vi "v6.vi"() -> ()   [LabVIEW 2025]
uses:
  <vilib>/Utility/miscctls.llb/LVDateTimeRec.ctl
  <vilib>/Platform/TimedLoop/XDataNode/timing_clust.ctl
  <vilib>/Platform/TimedLoop/XDataNode/nitl_modes.ctl
  <vilib>/Platform/TimedLoop/XDataNode/wakeup.ctl
  <vilib>/Analysis/3filter.llb/Filter Passband Type.ctl
  <vilib>/Instr/_visa.llb/VISA Configure Serial Port (Instr).vi
  <vilib>/Utility/inputDevices.llb/mouseAcquire.vi
  <vilib>/Analysis/3filter.llb/Butterworth Filter (DBL).vi
  <vilib>/Utility/file.llb/Write Delimited Spreadsheet (DBL).vi
  <vilib>/platform/TimedLoop/XDataNode/XDataNode.xnode
  <vilib>/Platform/TimedLoop/XDataNode/XDNodeRunTimeDep.lvlib
  <vilib>/Analysis/NI_AALPro.lvlib
  <vilib>/Analysis/NI_AALBase.lvlib
panel:
  out "erro_graus":dbl
  out "PV":dbl
  out "erro_abs_graus":dbl
  out "p_final":dbl
  out "array_frame_mov":i32[](array[numeric])
  out "array_mov":dbl[](array[numeric])
  out "TM_escre":string
  out "TM":i32
  out "ref":dbl
  out "velocidadepx":dbl[](array[numeric])
  out "referencia de endereco":path
  out "frames":i32[](array[numeric])
  out "TR":i32
  out "px_posicao":dbl[](array[numeric])
  out "t_max":dbl
  out "intervalo_preparacao":dbl
  out "intervalo_TR":dbl
  out "Vertical (cm/px)":dbl
  out "Horizontal (cm/px)":dbl
  out "INICIO_Cluter":T1
  out "INICIO":dbl format="%#.10g"
  out "ref_V_alvo":dbl
  out "ref_H_alvo":dbl
  out "ref_pont":dbl
  out "tentativa":i32
  out "cursor":picture
  in  "Tab Control":enum32{"Execucao", "Configuração"}(tab)
  out "tela":picture
  in  "Cor do ponteiro":u32(colorbox)=14421504
  in  "Cor_home":u32(colorbox)=197379
  in  "Horizontal (px)":dbl=1920.0
  in  "Horizontal (cm)":dbl=34.5
  in  "Raio_home":dbl=0.8
  in  "Horizontal_home":dbl=17.23
  in  "Vertical_home":dbl=20.0
  in  "Tamanho do ponteiro":dbl=0.3
  in  "Sincronizar com EEG":bool
  in  "Número de tentativas":i32=40
  in  "Digite aqui o endereço e nome do arquivo":string="C:\\bryan\\"
  in  "Vertical  (cm)":dbl=19.0
  in  "Vertical (px)":dbl=1080.0 format="%#_13g"
  in  "Horizontal_1":dbl=17.23
  in  "Vertical_1":dbl=23.0
  in  "Raio_1":dbl=0.5
  in  "Cor_1":u32(colorbox)=16775513
  in  "PORTA COM":refnum<visa-resource-name>
  in  "menor":dbl=2000.0 format="%#_13g"
  in  "preparacao 2":dbl=2000.0 format="%#_13g"
  in  "Tempo max  para fechar a tarefa":dbl=1500.0
  in  "FB":dbl=3000.0 format="%#_13g"
  in  "meta_tempo":dbl=250.0 format="%#_13g"
  out "home":picture
  # "100 h\n500 v"
  # "800 h\n100 v"
  # "Intervalo entre o prepara e vai"
  # "Tempo de preparação"
  # "Tempo de Feedback"
  # "Meta tempo"
  # "Home"
  # "Ponteiro"
  # "Para saber quantos cm preciso para um valor determinado de graus a percorre\n\n1. Divida o tamanho da tela vertical por 380 (ex.,19/380 = 0,05);\n2. Multiplique esse resultado pelo angulo de interesse (ex., 0,05*60 =3)"
  # "Posição do alvo"
  # "Horizontal"
  # "Raio"
  # "Vertical"
  # "Desenvolvido por Tércio Apolinário-Souza"
  # "Variability"
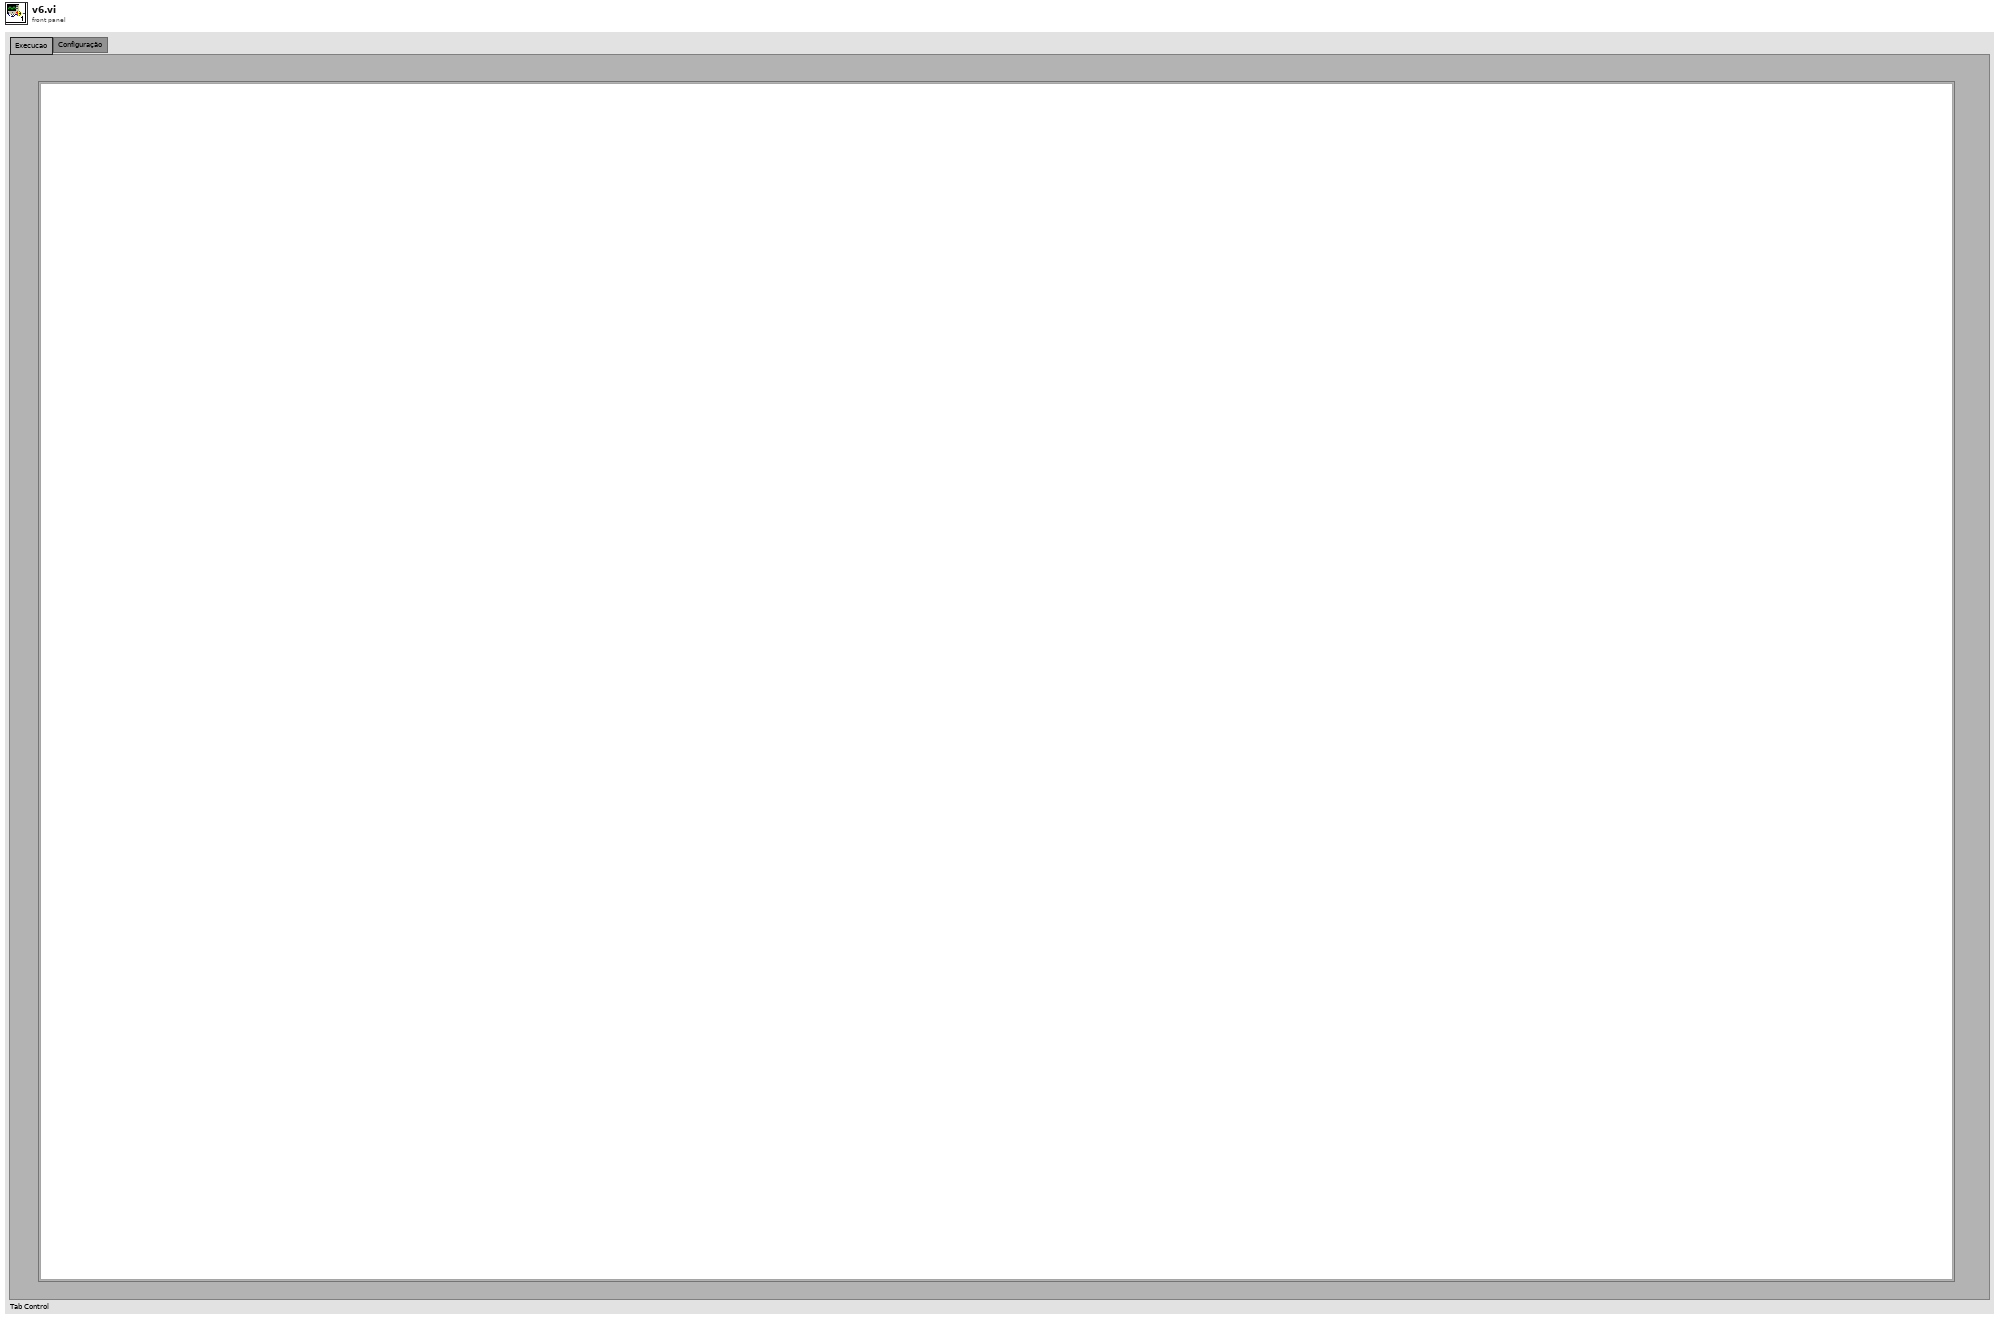
[diagram p1: front panel]
types:
  T1 = typedef "LVDateTimeRec.ctl" = cluster{"fractional second":dbl, "second":i32, "minute":i32, "hour":i32, "day of month":i32, "month":i32, "year":i32, "day of week":i32, "day of year":i32, "DST":i32}
  T2 = typedef "XDNodeRunTimeDep.lvlib/timing_clust.ctl" = cluster{"Expected End [f-1]":u64, "Actual End [f-1]":u64, "Finished Late? [f-1]":bool, "Expected End [i-1]":u64, "Actual End [i-1]":u64, "Finished Late? [i-1]":bool, "Expected Start [i]":u64, "Actual Start [i]":u64, "Expected Start [f]":u64, "Actual Start [f]":u64, "Source Name":string, "Structure Name":string, "Period":i64, "Deadline":i64, "Offset":i64, "Start":i64, "Priority":i32, "Timeout":i32, "Mode":T3, "Wakeup Reason":T4, "Error":errorcluster, "Source Type":string, "Secondary Source Type":string, "Global End Time":u64, "Global Start Time":u64, "Frame Duration":u64, "Iteration Duration":u64, "Assigned CPU":i32, "I/O Scan Engine Mode":u32}
  T3 = typedef "XDNodeRunTimeDep.lvlib/nitl_modes.ctl" = enum32{"No Change", "Process missed periods, maintain original phase", "Discard missed periods, maintain original phase", "Process missed periods, ignore original phase", "Discard missed periods, ignore original phase"}
  T4 = typedef "XDNodeRunTimeDep.lvlib/wakeup.ctl" = enum32{"Normal", "Aborted", "Asynchronous wakeup", "Timing source error", "Timed loop error", "Timeout"}
  T5 = typedef "NI_AALBase.lvlib/Filter Passband Type.ctl" = enum32{"Lowpass", "Highpass", "Bandpass", "Bandstop"}
  T6 = cluster{"button 1":bool, "button 2":bool, "button 3":bool, "button 4":bool}
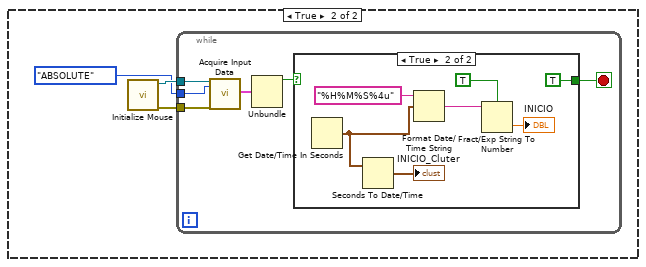
[diagram p2: hidden frame]
diagram:
  # "esquerda\ncima\ndireita\nbaixo"
  n1 = VISA Open(VISA resource name="PORTA COM") -> (VISA resource name=w21:refnum<visa-resource-name>, error out=w20:errorcluster)  [unwired: 4 in]
  n2 = VISA Close(VISA resource name=w21, error in (no error)=w20) -> (error out=w19:errorcluster)
  n3 = VISA Open(error in (no error)=w19, VISA resource name=w21) -> (VISA resource name=w18:refnum<visa-resource-name>, error out=w15:errorcluster)  [unwired: 3 in]
  n4 = for {
    N: "Número de tentativas" -> [_]
    tunnel: w18 -> [w38]
    tunnel: u32 9600 ("baud rate (9600)") -> [w37]
    tunnel: u16 8 ("data bits (8)") -> [w36]
    tunnel: w15 -> [w35]
    tunnel: [w30] -> w10 mode=indexing
    tunnel: [w29] -> w8 mode=indexing
    tunnel: [w28] -> w6 mode=indexing
    tunnel: [w27] -> w4 mode=indexing
    tunnel: [w26] -> w3 mode=indexing
    i -> [w40]
    n5 = call-poly "VISA Configure Serial Port"("VISA resource name"=w38, "baud rate (9600)"=w37, "data bits (8)"=w36, "error in (no error)"=w35) -> ("VISA resource name out"=w34:refnum<visa-resource-name>, "error out"=w33:errorcluster)  [unwired: 10 in]
    n6 = Increment(x=w40) -> (x+1=→"tentativa":i32)
    n7 = flat-sequence {
      tunnel: w40 -> [w44]
      tunnel: w34 -> [w42]
      tunnel: w33 -> [w43]
      tunnel: [w43] -> w32
      tunnel: [w42] -> w31
      tunnel: w32 -> [w74]
      tunnel: w31 -> [w75]
      tunnel: [w75] -> w25
      tunnel: [w74] -> w24
      tunnel: w25 -> [w94]
      tunnel: w24 -> [w93]
      tunnel: [w304] -> w30
      tunnel: [w301] -> w29
      tunnel: [w295] -> w28
      tunnel: [w290] -> w27
      tunnel: [w285] -> w26
      frame #0 {
        n8 = property on="TM_escre" class="Str"("Visible"=FALSE) -> ()  [unwired: 2 in, 2 out]
        n9 = Equal?(x=w44, y=0) -> (x = y?=w48:bool)
        n10 = And(x="Sincronizar com EEG", y=w48) -> (x .and. y?=w46:bool)
        n11 = case shown="False" w46 {
          frame False {
          }
          frame True {
            n12 = call <vilib>:"Initialize Mouse.vi"() -> ("error out"=w50:errorcluster, "device ID"=w51:refnum<k1>)  [unwired: 10 in]
            n13 = while {
              tunnel: w51 -> [w57]
              tunnel: w50 -> [w56]
              tunnel: enum16{"RELATIVE", "ABSOLUTE"}."ABSOLUTE" ("key mode") -> [w55]
              stop <- w53 stop-if-true
              n14 = call-poly <vilib>:"Acquire Input Data.vi"("device ID"=w57, "key mode"=w55, "error in (no error)"=w56) -> ("button info"=w54:T6)  [unwired: 13 in, 3 out]
              n15 = Unbundle(w54) -> ("button 1"=w52:bool)  [unwired: 3 out]
              n16 = case shown="True" w52 {
                tunnel: [_ TRUE] -> w53
                frame False {
                }
                frame True {
                  n17 = Get Date/Time In Seconds() -> (seconds since 1Jan1904=w59:timestamp)
                  n18 = Seconds To Date/Time(time stamp (now)=w59) -> (date time rec=→"INICIO_Cluter":T1)  [unwired: 1 in]
                  n19 = Format Date/Time String(time format string (%c)="%H%M%S%4u", seconds (now)=w59) -> (date/time string=w61:string)  [unwired: 1 in]
                  n20 = Fract/Exp String To Number(use system decimal point (T)=TRUE, string=w61) -> (number=→"INICIO":dbl)  [unwired: 2 in, 1 out]
                }
              }
            }
          }
        }
      }
      frame #1 {
        n21 = Quotient & Remainder(x="menor", y=5.0) -> (floor(x/y)=→"intervalo_TR":dbl)  [unwired: 1 out]
        n22 = Quotient & Remainder(x="preparacao 2", y=5.0) -> (floor(x/y)=→"intervalo_preparacao":dbl)  [unwired: 1 out]
        n23 = Divide(x="Vertical  (cm)", y="Vertical (px)") -> (x/y=→"Vertical (cm/px)":dbl)
        n24 = Divide(x="Horizontal (cm)", y="Horizontal (px)") -> (x/y=→"Horizontal (cm/px)":dbl)
        n25 = Quotient & Remainder(x="Tempo max  para fechar a tarefa", y=5.0) -> (floor(x/y)=→"t_max":dbl)  [unwired: 1 out]
      }
      frame #2 {
        n26 = node-c288(i64 5 ("Period")) -> (w92:T2)  [unwired: 3 in]
        n27 = timed-loop {
          tunnel: w94 -> [w152]
          tunnel: w93 -> [w151]
          timing: w92 -> [_]
          timing-out: [_] -> w91
          tunnel: [w144] -> w87
          tunnel: [w143] -> w86
          shift-right: [w124] -> w82
          shift-left: dbl[] [0.0] -> [w123]
          shift-right: [w122] -> w83
          shift-left: i32[] [0] -> [w121]
          i -> [w111]
          stop <- w145 stop-if-true
          # "Alvo"
          n28 = node-c288() -> ()  [unwired: 1 in, 1 out]
          n29 = VISA Read(VISA resource name=w152, byte count=u32 300, error in (no error)=w151) -> (VISA resource name out=w144:refnum<visa-resource-name>, read buffer=w153:string, error out=w143:errorcluster)  [unwired: 1 out]
          n30 = local read "Vertical_home"() -> (w142:dbl)
          n31 = local read "Vertical  (cm)"() -> (w169:dbl)
          n32 = local read "intervalo_TR"() -> (w128:dbl)
          n33 = local read "intervalo_preparacao"() -> (w119:dbl)
          n34 = local read "Horizontal (cm/px)"() -> (w161:dbl)
          n35 = local read "Horizontal_home"() -> (w141:dbl)
          n36 = local read "intervalo_TR"() -> (w120:dbl)
          n37 = local read "Raio_home"() -> (w140:dbl)
          n38 = local read "intervalo_preparacao"() -> (w106:dbl)
          n39 = local read "intervalo_preparacao"() -> (w126:dbl)
          n40 = local read "intervalo_preparacao"() -> (w131:dbl)
          n41 = local read "t_max"() -> (w129:dbl)
          n42 = Subtract(x=w169, y=w142) -> (x-y=w168:dbl)
          n43 = local read "intervalo_TR"() -> (w130:dbl)
          n44 = Spreadsheet String To Array(delimiter (Tab)=",", format string="%f", spreadsheet string=w153, array type (2D Dbl)=dbl[] []) -> (array=w154:dbl[])
          n45 = Add(x=w129, y=w128) -> (x+y=w127:dbl)
          n46 = Divide(x=w140, y=w161) -> (x/y=w166:dbl)
          n47 = Divide(x=w141, y=w161) -> (x/y=w171:dbl)
          n48 = Divide(x=w168, y=w161) -> (x/y=w146:dbl)
          n49 = Add(x=w120, y=w119) -> (x+y=w116:dbl)
          n50 = local read "Vertical  (cm)"() -> (w170:dbl)
          n51 = local read "Cor_home"() -> (w136:u32)
          n52 = local read "Vertical_1"() -> (w163:dbl)
          n53 = local read "Horizontal (cm/px)"() -> (w176:dbl)
          n54 = Add(x=w126, y=w127) -> (x+y=w125:dbl)
          n55 = Add(x=w131, y=w130) -> (x+y=w132:dbl)
          n56 = Index Array(array=w154) -> (element=w98:dbl)  [unwired: 1 in]
          n57 = Bundle(w171, w146) -> (w175:cluster{dbl, dbl})  [unwired: 1 in]
          n58 = Add(x=w116, y=2.0) -> (x+y=w115:dbl)
          n59 = Add(x=w106, y=2.0) -> (x+y=w110:dbl)
          n60 = local read "Horizontal_1"() -> (w165:dbl)
          n61 = Greater?(x=w111, y=w116) -> (0:w117:bool)
          n62 = Less?(x=w111, y=w115) -> (x < y?=w114:bool)
          n63 = Greater?(x=w111, y=w106) -> (0:w108:bool)
          n64 = Less?(x=w111, y=w110) -> (x < y?=w107:bool)
          n65 = Equal?(x=w125, y=w111) -> (x = y?=w145:bool)
          n66 = Greater?(x=w111, y=w131) -> (0:w134:bool)
          n67 = Less?(x=w111, y=w132) -> (x < y?=w133:bool)
          n68 = Subtract(x=w170, y=w163) -> (x-y=w167:dbl)
          n69 = Insert Into Array(array=w121, new element=w111) -> (w122:i32[])  [unwired: 1 in]
          n70 = Multiply(x=360.0, y=w98) -> (x*y=w149:dbl)
          n71 = And(x=w134, y=w133) -> ()  [unwired: 1 out]
          n72 = local read "Raio_1"() -> (w164:dbl)
          n73 = And(x=w117, y=w114) -> (x .and. y?=w113:bool)
          n74 = And(x=w108, y=w107) -> (x .and. y?=w109:bool)
          n75 = call <vilib>:"Draw Circle by Radius.vi"("color(black)"=w136, "fill?(F)"=TRUE, "pixel center"=w175, "radius"=w166) -> ("new picture"=w137:picture)  [unwired: 7 in]
          n76 = Divide(x=w165, y=w176) -> (x/y=w160:dbl)
          "ref_H_alvo" <- w160
          n77 = Divide(x=w167, y=w176) -> (x/y=w159:dbl)
          "ref_V_alvo" <- w159
          n78 = Divide(x=w149, y=1024.0) -> (x/y=w96:dbl)
          n79 = case shown="True" w113 {
            frame False {
            }
            frame True {
              # "Imperatus"
              n80 = call <vilib>:"Beep.vi"("use system alert? (T)"=FALSE, "duration (msec)"=u32 200, "frequency (Hz)"=u32 700) -> ()  [unwired: 9 in]
            }
          }
          n81 = case shown="True" w109 {
            frame False {
            }
            frame True {
              # "Warning"
              n82 = call <vilib>:"Beep.vi"("use system alert? (T)"=FALSE, "duration (msec)"=u32 200, "frequency (Hz)"=u32 500) -> ()  [unwired: 9 in]
            }
          }
          n83 = local write "home"(w137) -> ()
          n84 = Divide(x=w164, y=w176) -> (x/y=w178:dbl)
          n85 = local read "Horizontal (px)"() -> (w104:dbl)
          n86 = local read "Vertical (px)"() -> (w105:dbl)
          n87 = local read "Tamanho do ponteiro"() -> (w139:dbl)
          n88 = local read "Horizontal (cm/px)"() -> (w173:dbl)
          n89 = Bundle(w160, w159) -> (w99:cluster{dbl, dbl})  [unwired: 1 in]
          n90 = Divide(x=w96, y=380.0) -> (x/y=w97:dbl)
          n91 = local read "Cor_1"() -> (w162:u32)
          n92 = local read "Cor do ponteiro"() -> (w135:u32)
          n93 = Multiply(x=w97, y=w105) -> (x*y=w95:dbl)
          n94 = Quotient & Remainder(x=w104, y=2.0) -> (floor(x/y)=w102:dbl)  [unwired: 1 out]
          n95 = Divide(x=w139, y=w173) -> (x/y=w172:dbl)
          "ref_pont" <- w172
          n96 = Insert Into Array(array=w123, new element=w95) -> (w124:dbl[])  [unwired: 1 in]
          n97 = call <vilib>:"Draw Circle by Radius.vi"("color(black)"=w162, "fill?(F)"=TRUE, "pixel center"=w99, "radius"=w178, "picture"=w137) -> ("new picture"=w138:picture)  [unwired: 6 in]
          n98 = Bundle(w102, w95) -> (w180:cluster{dbl, dbl})  [unwired: 1 in]
          n99 = local write "cursor"(w138) -> ()
          n100 = call <vilib>:"Draw Circle by Radius.vi"("color(black)"=w135, "fill?(F)"=TRUE, "pixel center"=w180, "radius"=w172, "picture"=w138) -> ("new picture"=w100:picture)  [unwired: 6 in]
          n101 = call <vilib>:"Draw Circle by Radius.vi"("picture"=w100) -> ("new picture"=w101:picture)  [unwired: 10 in]
          n102 = local write "tela"(w101) -> ()
          n103 = node-c288() -> ()  [unwired: 1 in, 1 out]
        }
        "px_posicao" <- w82
        "frames" <- w83
        n104 = node-c288(w91) -> ()  [unwired: 1 out]
        n105 = VISA Clear(VISA resource name=w87, error in (no error)=w86) -> (VISA resource name out=w89:refnum<visa-resource-name>, error out=w88:errorcluster)
        n106 = VISA Close(VISA resource name=w89, error in (no error)=w88) -> ()  [unwired: 1 out]
      }
      frame #3 {
        # "Filtro"
        # "Filtro"
        n107 = call <vilib>:"Draw Circle by Radius.vi"() -> ("new picture"=w213:picture)  [unwired: 11 in]
        n108 = local write "tela"(w213) -> ()
        n109 = local read "px_posicao"() -> (w200:dbl[])
        n110 = Wait (ms)(milliseconds to wait=u32 10) -> ()  [unwired: 1 out]
        n111 = call-poly <vilib>:"Butterworth Filter.vi"("order"=2, "filter type"=Filter_Passband_Type."Lowpass", "low cutoff freq: fl"=12.0, "sampling freq: fs"=200.0, "X"=w200) -> ("Filtered X"=w208:dbl[])  [unwired: 3 in, 1 out]
        n112 = call <vilib>:"Derivative x(t).vi"("dt"=0.01, "Initial Condition"=dbl[] [0.0], "X"=w208) -> ("dX/dt"=w201:dbl[])  [unwired: 7 in, 1 out]
        n113 = call-poly <vilib>:"Butterworth Filter.vi"("order"=2, "filter type"=Filter_Passband_Type."Lowpass", "low cutoff freq: fl"=12.0, "sampling freq: fs"=100.0, "X"=w201) -> ("Filtered X"=w195:dbl[])  [unwired: 3 in, 1 out]
        n114 = Array Size(array=w195) -> (size(s)=w198:i32)
        n115 = Subtract(x=w198, y=1) -> (x-y=w196:i32)
        n116 = Array Subset(array=w195, index=0, length=w196) -> (→"velocidadepx":dbl[])
      }
      frame #4 {
        n117 = while {
          tunnel: [w220] -> w215
          tunnel: [w217] -> w216
          i -> [w220]
          stop <- w218 stop-if-true
          n118 = local read "intervalo_preparacao"() -> (w225:dbl)
          n119 = local read "velocidadepx"() -> (w227:dbl[])
          n120 = local read "intervalo_TR"() -> (w226:dbl)
          n121 = Add(x=w226, y=w225) -> (x+y=w217:dbl)
          n122 = Array Size(array=w227) -> (size(s)=w219:i32)
          n123 = Array Subset(array=w227, index=w217, length=w219) -> (w224:dbl[])
          n124 = Absolute Value(x=w224) -> (abs(x)=w223:dbl[])
          n125 = Greater?(x=w220, y=w219) -> (0:w221:bool)
          n126 = Index Array(array=w223, index=w220) -> (element=w231:dbl)
          n127 = Array Max & Min(array=w223) -> (max value=w230:dbl)  [unwired: 3 out]
          "PV" <- w230
          n128 = Multiply(x=w230, y=0.2) -> (x*y=w228:dbl)
          "ref" <- w228
          n129 = Greater?(x=w231, y=w228) -> (0:w222:bool)
          n130 = Or(x=w222, y=w221) -> (x .or. y?=w218:bool)
        }
        n131 = Add(x=w216, y=w215) -> (x+y=→"TR":dbl)
      }
      frame #5 {
        n132 = while {
          tunnel: [w239] -> w232
          shift-right: [w241] -> w235
          shift-left: dbl[] [0.0] -> [w240]
          shift-right: [w238] -> w233
          shift-left: i32[] [0] -> [w237]
          i -> [w239]
          stop <- w243 stop-if-true
          n133 = local read "velocidadepx"() -> (w250:dbl[])
          n134 = Array Size(array=w250) -> (size(s)=w246:i32)
          n135 = local read "TR"() -> (w251:i32)
          n136 = Array Subset(array=w250, index=w251, length=w246) -> (w249:dbl[])
          n137 = Absolute Value(x=w249) -> (abs(x)=w247:dbl[])
          n138 = Greater?(x=w239, y=w246) -> (0:w245:bool)
          n139 = Insert Into Array(array=w237, new element=w239) -> (w238:i32[])  [unwired: 1 in]
          n140 = Index Array(array=w247, index=w239) -> (element=w242:dbl)
          n141 = local read "ref"() -> (w248:dbl)
          n142 = Insert Into Array(array=w240, new element=w242) -> (w241:dbl[])  [unwired: 1 in]
          n143 = Less?(x=w242, y=w248) -> (x < y?=w244:bool)
          n144 = Or(x=w245, y=w244) -> (x .or. y?=w243:bool)
        }
        "TM" <- w232
        "array_mov" <- w235
        "array_frame_mov" <- w233
      }
      frame #6 {
        w262 = ".xls" ("string")
        n145 = local read "px_posicao"() -> (w284:dbl[])
        n146 = local read "Digite aqui o endereço e nome do arquivo"() -> (w265:string)
        n147 = local read "TR"() -> (w283:i32)
        n148 = local read "TM"() -> (w277:i32)
        n149 = Array Subset(array=w284, index=w283, length=w277) -> (w279:dbl[])
        n150 = Array Size(array=w279) -> (size(s)=w282:i32)
        n151 = local read "Vertical (px)"() -> (w260:dbl)
        n152 = local read "tentativa"() -> (w268:i32)
        n153 = Subtract(x=w282, y=1) -> (x-y=w280:i32)
        n154 = local read "velocidadepx"() -> (w254:dbl[])
        n155 = local read "px_posicao"() -> (w258:dbl[])
        n156 = Index Array(array=w279, index=w280) -> (element=→"p_final":dbl)
        n157 = Concatenate Strings(w265, w262) -> (w263:string)
        n158 = Concatenate Strings(w265, "_tentativa_" ("string")) -> (w266:string)
        n159 = Format Into String(w268) -> (resulting string=w267:string)  [unwired: 3 in, 1 out]
        n160 = Divide(x=380.0, y=w260) -> (x/y=w255:dbl)
        n161 = local read "frames"() -> (w273:i32[])
        n162 = Multiply(x=w258, y=w255) -> (x*y=w257:dbl[])
        n163 = Multiply(x=w254, y=w255) -> (x*y=w253:dbl[])
        n164 = Concatenate Strings(w266, w267) -> (w269:string)
        n165 = String To Path(string=w263) -> (path=→"referencia de endereco":path)
        n166 = call "Convert to Dynamic Data6"("Array"=w258) -> ("Dynamic Data Type"=w275:dynamicdata)  [unwired: 3 in]
        n167 = call "Convert to Dynamic Data5"("Array"=w254) -> ("Dynamic Data Type"=w276:dynamicdata)  [unwired: 3 in]
        n168 = call "Convert to Dynamic Data2"("Array"=w273) -> ("Dynamic Data Type"=w274:dynamicdata)  [unwired: 3 in]
        n169 = call "Convert to Dynamic Data3"("Array"=w257) -> ("Dynamic Data Type"=w256:dynamicdata)  [unwired: 3 in]
        n170 = call "Convert to Dynamic Data4"("Array"=w253) -> ("Dynamic Data Type"=w252:dynamicdata)  [unwired: 3 in]
        n171 = Concatenate Strings(w269, w262) -> (w270:string)
        n172 = String To Path(string=w270) -> (path=w271:path)
        n173 = Merge Signals(w274, w275, w276, w256, w252) -> (w272:dynamicdata)
        n174 = call "Salvar em xls"("Signals"=w272, "Filename"=w271) -> ()  [unwired: 15 in, 3 out]
      }
      frame #7 {
        n175 = local read "TM"() -> (w317:i32)
        n176 = property on="TM_escre" class="Str"("Visible"=TRUE) -> ()  [unwired: 2 in, 2 out]
        n177 = Wait (ms)(milliseconds to wait="FB") -> ()  [unwired: 1 out]
        n178 = Multiply(x=w317, y=5) -> (x*y=w318:i32)
        n179 = local read "ref_V_alvo"() -> (w300:dbl)
        n180 = local read "intervalo_preparacao"() -> (w308:dbl)
        n181 = local read "p_final"() -> (w299:dbl)
        n182 = Number To Decimal String(number="meta_tempo") -> (decimal integer string=w312:string)  [unwired: 1 in]
        n183 = Number To Decimal String(number=w318) -> (decimal integer string=w309:string)  [unwired: 1 in]
        n184 = local read "intervalo_TR"() -> (w307:dbl)
        n185 = local read "Vertical (px)"() -> (w297:dbl)
        n186 = Concatenate Strings(w312, "\r\n", w309) -> (w311:string)
        n187 = Subtract(x=w300, y=w299) -> (x-y=w287:dbl)
        n188 = local read "Vertical (px)"() -> (w293:dbl)
        n189 = local write "TM_escre"(w311) -> ()
        n190 = Add(x=w308, y=w307) -> (x+y=w289:dbl)
        n191 = Absolute Value(x=w287) -> (abs(x)=w296:dbl)
        n192 = Divide(x=380.0 ("y"), y=w297) -> (x/y=w286:dbl)
        n193 = local read "TR"() -> (w288:i32)
        n194 = Multiply(x=w296, y=w286) -> (x*y=w295:dbl)
        "erro_abs_graus" <- w295
        n195 = Multiply(x=w287, y=w286) -> (x*y=w285:dbl)
        "erro_graus" <- w285
        n196 = Divide(x=380.0, y=w293) -> (x/y=w292:dbl)
        n197 = Subtract(x=w288, y=w289) -> (x-y=w305:dbl)
        n198 = local read "PV"() -> (w291:dbl)
        n199 = local read "TM"() -> (w303:i32)
        n200 = Multiply(x=w292, y=w291) -> (x*y=w290:dbl)
        n201 = Multiply(x=w303, y=5) -> (x*y=w301:i32)
        n202 = Multiply(x=w305, y=5.0) -> (x*y=w304:dbl)
      }
    }
  }
  n203 = call "Convert to Dynamic Data9"("Array"=w10) -> ("Dynamic Data Type"=w9:dynamicdata)  [unwired: 3 in]
  n204 = call "Convert to Dynamic Data10"("Array"=w8) -> ("Dynamic Data Type"=w7:dynamicdata)  [unwired: 3 in]
  n205 = call "Convert to Dynamic Data11"("Array"=w6) -> ("Dynamic Data Type"=w5:dynamicdata)  [unwired: 3 in]
  n206 = call "Convert to Dynamic Data7"("Array"=w3) -> ("Dynamic Data Type"=w1:dynamicdata)  [unwired: 3 in]
  n207 = call "Convert to Dynamic Data"("Array"=w4) -> ("Dynamic Data Type"=w2:dynamicdata)  [unwired: 3 in]
  n208 = Merge Signals(w9, w7, w5, w1, w2) -> (w11:dynamicdata)
  n209 = call "Dados Brutos"("Signals"=w11) -> ("Table"=w13:string[][])  [unwired: 4 in, 6 out]
  n210 = Fract/Exp String To Number(string=w13) -> (number=w14:dbl[][])  [unwired: 3 in, 1 out]
  n211 = call-poly <vilib>:"Write Delimited Spreadsheet.vi"("format (%.3f)"="%.3f", "2D data"=w14) -> ()  [unwired: 12 in, 2 out]
